vi "LB_FocusIndex_Tests.vi"(11 "error in":errorcluster) -> (15 "error out":errorcluster)   [LabVIEW 2016, in "DronaTest.lvlib"]
uses:
  DronaTest.lvlib
  APIs/Stimulus/ControlValue/SetValueAuto.vi
  APIs/Stimulus/ControlValue/Controls/Listbox/SetValueByItemIndex.vi
  APIs/Assert/AssertControlValue/Controls/Listbox/AssertValueByFocusIndex.vi
  <vilib>/addons/_JKI Toolkits/Caraya/classes/Assert/Assert Error.vi
  <vilib>/addons/_JKI Toolkits/Caraya/classes/Assert/Assert Equal Value_Variant.vi
  <vilib>/addons/_JKI Toolkits/Caraya/classes/Test/Test.lvclass
  Drona.lvlib
  <vilib>/SLL Toolkit/SLL Debug/SLL Debug.lvlib
  APIs/Stimulus/ControlValue/Controls/Listbox/StimulusListbox.lvlib
  <vilib>/addons/_JKI Toolkits/Caraya/classes/Assert/Assert.lvclass
  APIs/Assert/AssertControlValue/Controls/Listbox/AssertListbox.lvlib
  APIs/Stimulus/ControlValue/ControlValue.lvlib
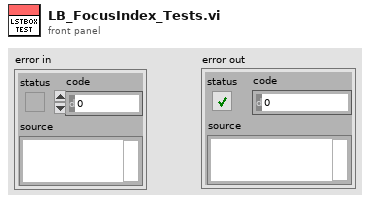
[diagram p1: front panel]
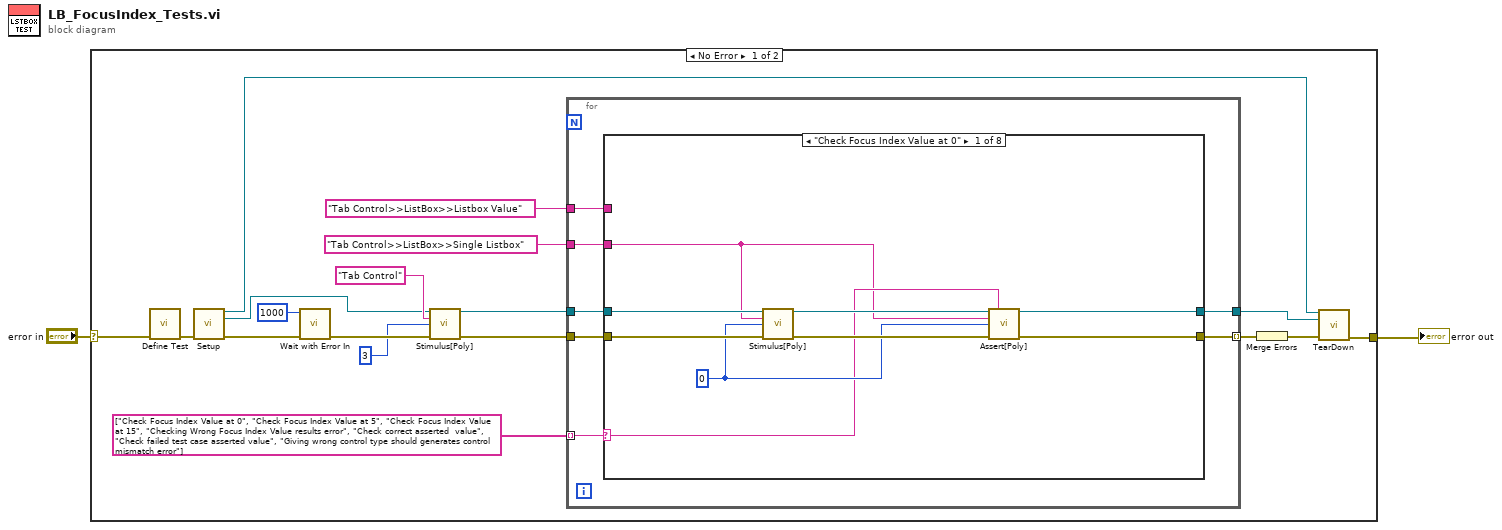
[diagram p0: block diagram]
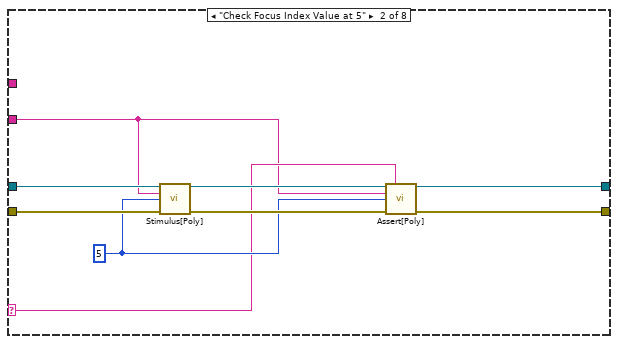
[diagram p2: hidden frame]
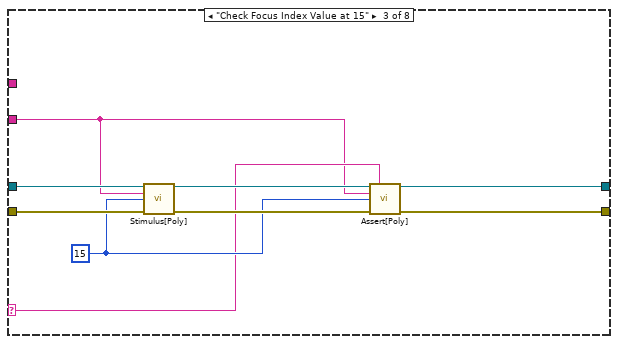
[diagram p3: hidden frame]
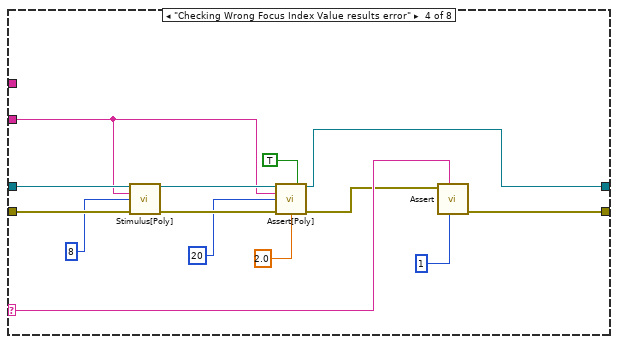
[diagram p4: hidden frame]
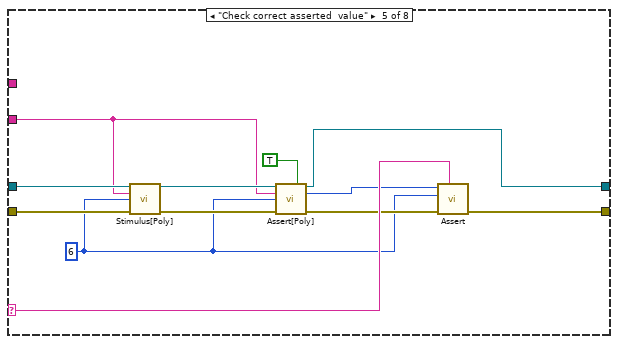
[diagram p5: hidden frame]
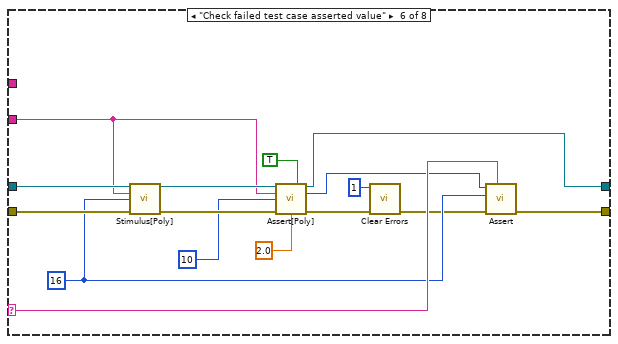
[diagram p6: hidden frame]
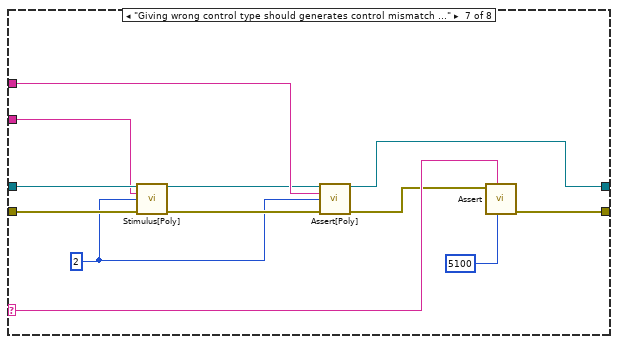
[diagram p7: hidden frame]
diagram:
  n1 = case shown="No Error" "error in" {
    selector: "error in" -> [w20 w111]
    tunnel: [w3 w111] -> w1
    frame No Error {
      n2 = call <vilib>:"Define Test.vi"("error in (no error)"=w20) -> ("error out"=w9:errorcluster)  [unwired: 9 in, 1 out]
      n3 = call "Setup.vi"("error in"=w9) -> ("Application Ref"=w5:refnum<vi>, "VI out"=w7:refnum<vi>, "error out"=w8:errorcluster)  [unwired: 12 in]
      n4 = call <vilib>:"Wait with Error In.vi"("error in (no error)"=w8, "milliseconds to wait"=u32 1000) -> ("error out"=w18:errorcluster)  [unwired: 9 in]
      n5 = call-poly "Stimulus[Poly].vi"("VI Reference In"=w7, "Control Path"="Tab Control", "Value (Signaling)"=3, "error in"=w18) -> ("VI Reference Out"=w14:refnum<vi>, "error out"=w17:errorcluster)  [unwired: 10 in]
      n6 = for {
        tunnel: w14 -> [w26]
        tunnel: "Tab Control>>ListBox>>Single Listbox" ("Control Path") -> [w25]
        tunnel: "Tab Control>>ListBox>>Listbox Value" ("Control Path") -> [w24]
        tunnel: string[] ["Check Focus Index Value at 0", "Check Focus Index Value at 5", "Check Focus Index Value at 15", "Checking Wrong Focus Index Value results error", "Check correct asserted  value", "Check failed test case asserted value", "Giving wrong control type should generates control mismatch error"] -> [w22] mode=indexing
        tunnel: [w21] -> w4
        tunnel: w17 -> [w27]
        tunnel: [w23] -> w10 mode=indexing
        n7 = case shown="\"Check Focus Index Value at 0\"" w22 {
          selector: w22 -> [w29 w38 w47 w67 w79 w95 w107 _]
          tunnel: w27 -> [w36 w45 w54 w65 w78 w94 w102 w110]
          tunnel: w26 -> [w35 w44 w53 w64 w77 w93 w100 w109]
          tunnel: w25 -> [w28 w37 w46 w60 w74 w90 w98 _]
          tunnel: w24 -> [_ _ _ _ _ _ w104 _]
          tunnel: [w31 w40 w49 w68 w80 w96 w108 w110] -> w23
          tunnel: [w30 w39 w48 w58 w73 w89 w103 w109] -> w21
          frame "Check Focus Index Value at 0" {
            w32 = 0 ("Item Index")
            n8 = call-poly "Stimulus[Poly].vi"("VI Reference In"=w35, "Control Path"=w28, "Item Index"=w32, "Error In"=w36) -> ("VI Reference Out"=w33:refnum<vi>, "Error Out"=w34:errorcluster)  [unwired: 10 in]
            n9 = call-poly "Assert[Poly].vi"("VI Reference In"=w33, "Test Label"=w29, "Control Path"=w28, "Focus Index"=w32, "Error In"=w34) -> ("VI Reference Out"=w30:refnum<vi>, "Error Out"=w31:errorcluster)  [unwired: 8 in, 1 out]
          }
          frame "Check Focus Index Value at 5" {
            w41 = 5 ("Item Index")
            n10 = call-poly "Stimulus[Poly].vi"("VI Reference In"=w44, "Control Path"=w37, "Item Index"=w41, "Error In"=w45) -> ("VI Reference Out"=w42:refnum<vi>, "Error Out"=w43:errorcluster)  [unwired: 10 in]
            n11 = call-poly "Assert[Poly].vi"("VI Reference In"=w42, "Test Label"=w38, "Control Path"=w37, "Focus Index"=w41, "Error In"=w43) -> ("VI Reference Out"=w39:refnum<vi>, "Error Out"=w40:errorcluster)  [unwired: 8 in, 1 out]
          }
          frame "Check Focus Index Value at 15" {
            w50 = 15 ("Item Index")
            n12 = call-poly "Stimulus[Poly].vi"("VI Reference In"=w53, "Control Path"=w46, "Item Index"=w50, "Error In"=w54) -> ("VI Reference Out"=w51:refnum<vi>, "Error Out"=w52:errorcluster)  [unwired: 10 in]
            n13 = call-poly "Assert[Poly].vi"("VI Reference In"=w51, "Test Label"=w47, "Control Path"=w46, "Focus Index"=w50, "Error In"=w52) -> ("VI Reference Out"=w48:refnum<vi>, "Error Out"=w49:errorcluster)  [unwired: 8 in, 1 out]
          }
          frame "Checking Wrong Focus Index Value results error" {
            n14 = call-poly "Stimulus[Poly].vi"("VI Reference In"=w64, "Control Path"=w60, "Item Index"=8, "Error In"=w65) -> ("VI Reference Out"=w61:refnum<vi>, "Error Out"=w62:errorcluster)  [unwired: 10 in]
            n15 = call-poly "Assert[Poly].vi"("VI Reference In"=w61, "Assert Only? (F)"=TRUE, "Control Path"=w60, "Focus Index"=20 ("Item Index"), "Error In"=w62, "Timeout(5 sec)"=2.0) -> ("VI Reference Out"=w58:refnum<vi>, "Error Out"=w57:errorcluster)  [unwired: 7 in, 1 out]
            n16 = call-poly <vilib>:"Assert.vi"("error code (1)"=1, "Label"=w67, "Error?"=w57) -> ("error out"=w68:errorcluster)  [unwired: 7 in, 1 out]
          }
          frame "Check correct asserted  value" {
            w70 = 6 ("Item Index")
            n17 = call-poly "Stimulus[Poly].vi"("VI Reference In"=w77, "Control Path"=w74, "Item Index"=w70, "Error In"=w78) -> ("VI Reference Out"=w75:refnum<vi>, "Error Out"=w76:errorcluster)  [unwired: 10 in]
            n18 = call-poly "Assert[Poly].vi"("VI Reference In"=w75, "Assert Only? (F)"=TRUE, "Control Path"=w74, "Focus Index"=w70, "Error In"=w76) -> ("VI Reference Out"=w73:refnum<vi>, "Asserted Value"=w71:i32, "Error Out"=w72:errorcluster)  [unwired: 8 in]
            n19 = call-poly <vilib>:"Assert.vi"("Label"=w79, "error in (no error)"=w72, "Y"=w70, "X"=w71) -> ("error out"=w80:errorcluster)  [unwired: 6 in, 1 out]
          }
          frame "Check failed test case asserted value" {
            w87 = 16 ("Item Index")
            n20 = call-poly "Stimulus[Poly].vi"("VI Reference In"=w93, "Control Path"=w90, "Item Index"=w87, "Error In"=w94) -> ("VI Reference Out"=w91:refnum<vi>, "Error Out"=w92:errorcluster)  [unwired: 10 in]
            n21 = call-poly "Assert[Poly].vi"("VI Reference In"=w91, "Assert Only? (F)"=TRUE, "Control Path"=w90, "Focus Index"=10 ("Item Index"), "Error In"=w92, "Timeout(5 sec)"=2.0) -> ("VI Reference Out"=w89:refnum<vi>, "Asserted Value"=w81:i32, "Error Out"=w88:errorcluster)  [unwired: 7 in]
            n22 = call <vilib>:"Clear Errors.vi"("error in (no error)"=w88, "specific error code to clear (0: all)"=1) -> ("error out"=w83:errorcluster)  [unwired: 4 in, 1 out]
            n23 = call-poly <vilib>:"Assert.vi"("Label"=w95, "error in (no error)"=w83, "Y"=w87, "X"=w81) -> ("error out"=w96:errorcluster)  [unwired: 6 in, 1 out]
          }
          frame "Giving wrong control type should generates control mismatch error" {
            w97 = 2 ("Item Index")
            n24 = call-poly "Stimulus[Poly].vi"("VI Reference In"=w100, "Control Path"=w98, "Item Index"=w97, "Error In"=w102) -> ("VI Reference Out"=w99:refnum<vi>, "Error Out"=w101:errorcluster)  [unwired: 10 in]
            n25 = call-poly "Assert[Poly].vi"("VI Reference In"=w99, "Control Path"=w104, "Focus Index"=w97, "Error In"=w101) -> ("VI Reference Out"=w103:refnum<vi>, "Error Out"=w105:errorcluster)  [unwired: 9 in, 1 out]
            n26 = call-poly <vilib>:"Assert.vi"("error code (1)"=5100, "Label"=w107, "Error?"=w105) -> ("error out"=w108:errorcluster)  [unwired: 7 in, 1 out]
          }
          frame Default {
          }
        }
      }
      n27 = Merge Errors(w10) -> (w6:errorcluster)
      n28 = call "TearDown.vi"("Application Ref"=w5, "VI in"=w4, "error in (no error)"=w6) -> ("error out"=w3:errorcluster)  [unwired: 12 in]
    }
    frame Error {
    }
  }
  "error out" <- w1
